vi "VIH Utility - VISRV - Get Datatype Terminal Icon.vi"(8 "error in":errorcluster, 10 "Indicator":bool, 11 "Datatype":variant) -> (0 "error out":errorcluster, 3 "Icon":picture)   [LabVIEW 2014]
doc: "::: VI Helpeks :::\nCopyright (c) 2000-2026 Konstantin Shifershteyn. All rights reserved."
panel:
  # "VI Helpeks\nCopyright (c) 2012-2026 Konstantin Shifershteyn"
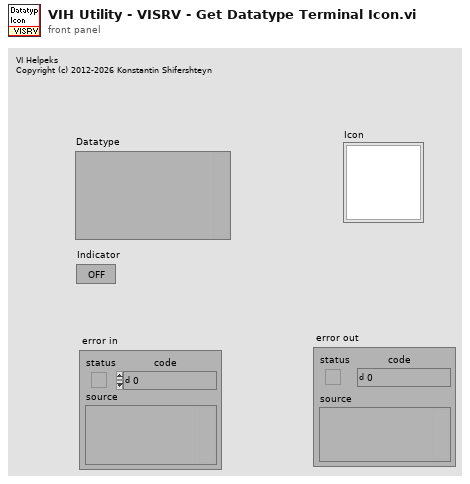
[diagram p1: front panel]
types:
  T1 = typedef "imagedata.ctl" = cluster{"image type":i32, "image depth":i32, "image":u8[], "mask":u8[], "colors":u32[], "Rectangle":cluster{"left":i16, "top":i16, "right":i16, "bottom":i16}}
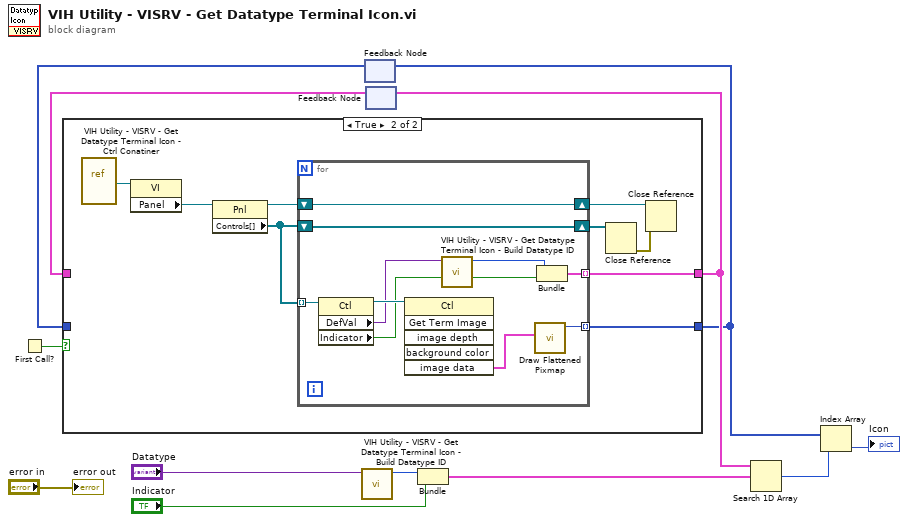
[diagram p0: block diagram]
diagram:
  n1 = First Call?() -> (First Call?: T/F=w12:bool)
  n2 = call "VIH Utility - VISRV - Get Datatype Terminal Icon - Build Datatype ID.vi"("Datatype"="Datatype") -> ("Type ID"=w1:u64)  [unwired: 10 in]
  n3 = feedback #1() -> (w10:picture[])  [unwired: 1 in]
  n4 = feedback #2() -> (w11:cluster{"Type ID":u64, "Indicator":bool}[])  [unwired: 1 in]
  n5 = case shown="True" w12 {
    tunnel: [w14 w16] -> w7
    tunnel: w11 -> [w14 _]
    tunnel: [w13 w15] -> w5
    tunnel: w10 -> [w13 _]
    frame False {
    }
    frame True {
      n6 = vi-ref "VIH Utility - VISRV - Get Datatype Terminal Icon - Ctrl Conatiner.vi"() -> (w23:refnum<vi>)
      n7 = property class="VI"(reference=w23) -> ("Panel"=w22:refnum<vi>)  [unwired: 1 in, 2 out]
      n8 = property class="Pnl"(reference=w22) -> (reference out=w19:refnum<vi>, "Controls[]"=w21:refnum<vi>[])  [unwired: 1 in, 1 out]
      n9 = for {
        tunnel: w21 -> [w33] mode=indexing
        tunnel: [w30] -> w15 mode=indexing
        tunnel: [w28] -> w16 mode=indexing
        shift-right: [w27] -> w20
        shift-left: w21 -> [w27]
        shift-right: [w26] -> w18
        shift-left: w19 -> [w26]
        n10 = property class="Ctl"(reference=w33) -> (reference out=w32:refnum<vi>, "DefVal"=w25:variant, "Indicator"=w29:bool)  [unwired: 1 in, 1 out]
        n11 = invoke class="Ctl" method="Get Term Image"(reference=w32) -> ("image data"=w31:T1)  [unwired: 5 in, 5 out]
        n12 = call "VIH Utility - VISRV - Get Datatype Terminal Icon - Build Datatype ID.vi"("Datatype"=w25) -> ("Type ID"=w24:u64)  [unwired: 10 in]
        n13 = call <vilib>:"Draw Flattened Pixmap.vi"("image data"=w31) -> ("new picture"=w30:picture)  [unwired: 8 in]
        n14 = Bundle("Type ID"=w24, "Indicator"=w29) -> (w28:cluster{"Type ID":u64, "Indicator":bool})  [unwired: 1 in]
      }
      n15 = Close Reference(reference=w20) -> (error out=w17:errorcluster)  [unwired: 1 in]
      n16 = Close Reference(reference=w18, error in (no error)=w17) -> ()  [unwired: 1 out]
    }
  }
  n17 = feedback-in #1(w5) -> ()
  n18 = feedback-in #2(w7) -> ()
  n19 = Bundle("Type ID"=w1, "Indicator"="Indicator") -> (w8:cluster{"Type ID":u64, "Indicator":bool})  [unwired: 1 in]
  n20 = Search 1D Array(1D array=w7, element=w8) -> (index of element=w6:i32)  [unwired: 1 in]
  n21 = Index Array(array=w5, index=w6) -> (element=→"Icon":picture)
  "error out" <- "error in"
